vi "MC AOTF Engine.vi"(0 "Notifier Name":string, 11 "Ports (Unused)":string[](array[string])) -> ()   [LabVIEW 2016]
uses:
  AOTF Controls/AOTF Notifier Element.ctl
  AOTF Controls/AOTF Actions.ctl
  AOTF Controls/AOTF Lines Lines Control.ctl
  <vilib>/ULx/Create Channel.llb/ULx Create Channel (DO-Digital Output).vi
  <vilib>/ULx/Write.llb/ULx Write (Digital Bool 1Line 1Point).vi
  <vilib>/ULx/Create Channel.llb/ULx Create Channel (AO-Voltage-Basic).vi
  <vilib>/ULx/Write.llb/ULx Write (Analog 1D DBL 1Chan 1Samp).vi
panel:
  in  "Blank":bool
  in  "Quit":bool
  in  "500":dbl(slide) scale=0.0..100.0
  in  "642":dbl(slide) scale=0.0..100.0
  in  "560":dbl(slide) scale=0.0..100.0
  in  "488":dbl(slide) scale=0.0..100.0
  in  "405":dbl(slide) scale=0.0..100.0
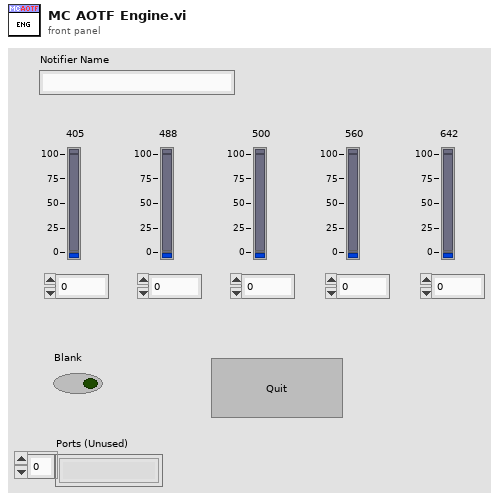
[diagram p1: front panel]
types:
  T1 = typedef "AOTF Lines Lines Control.ctl" = cluster{"Wavelength":u16[], "AO Line":string[]}
  T2 = typedef "AOTF Notifier Element.ctl" = cluster{"AOTF Action":T3, "Laser Line":string, "Power (%)":dbl, "Beam Blank On/Off":bool, "Line On/Off":bool, "Error":errorcluster, "Wavelengths (nm)":string[]}
  T3 = typedef "AOTF Actions.ctl" = enum16{"Error Check", "Blank", "Line On/Off", "Set Power", "Status", "Quit"}
  T4 = enum32{"Invalid", "Standard", "Closed", "Hidden", "Minimized", "Maximized"}
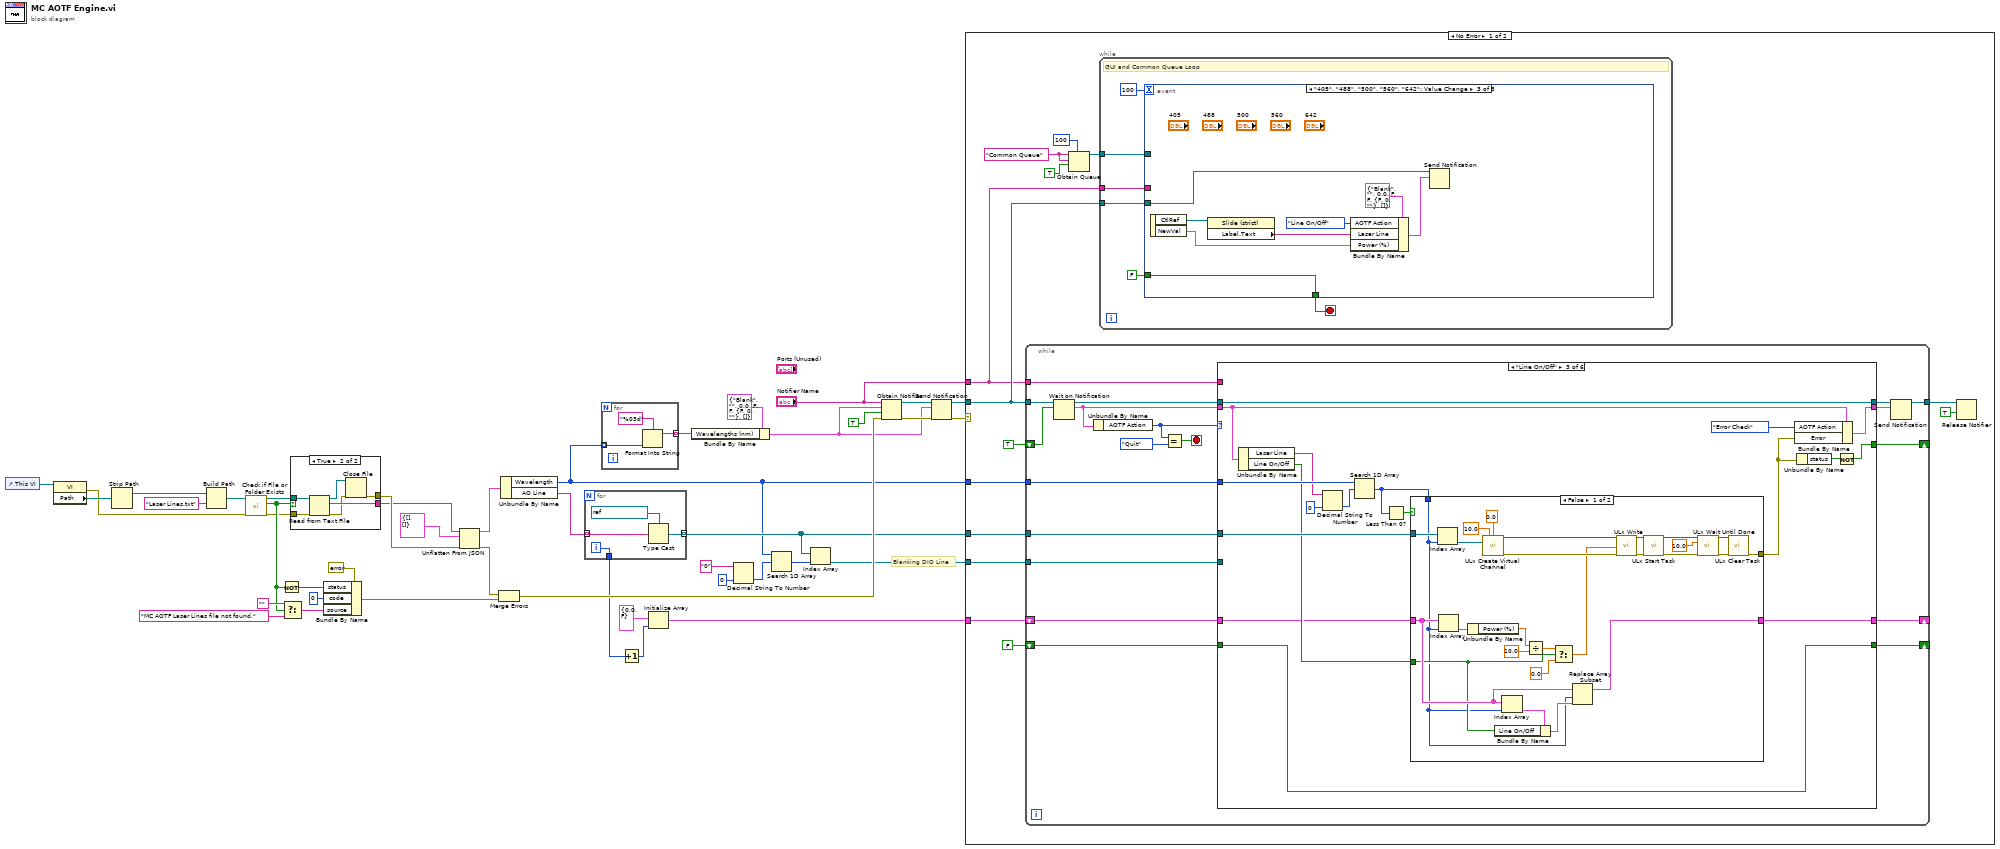
[diagram p0: block diagram]
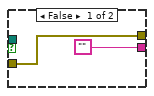
[diagram p2: hidden frame]
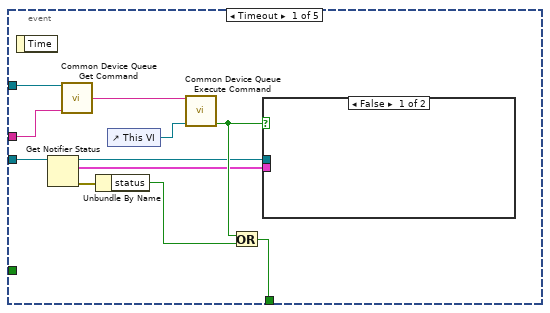
[diagram p3: hidden frame]
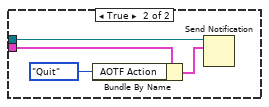
[diagram p4: hidden frame]
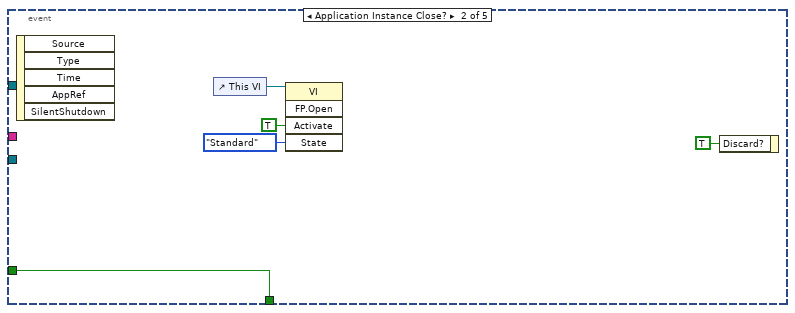
[diagram p5: hidden frame]
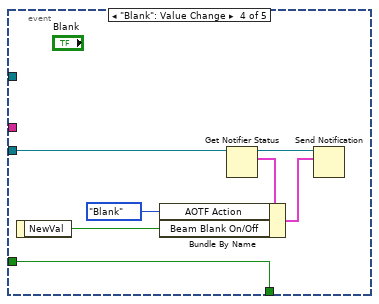
[diagram p6: hidden frame]
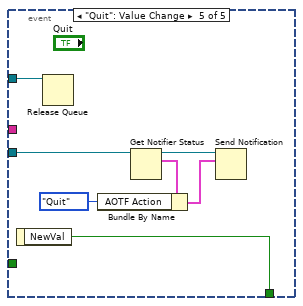
[diagram p7: hidden frame]
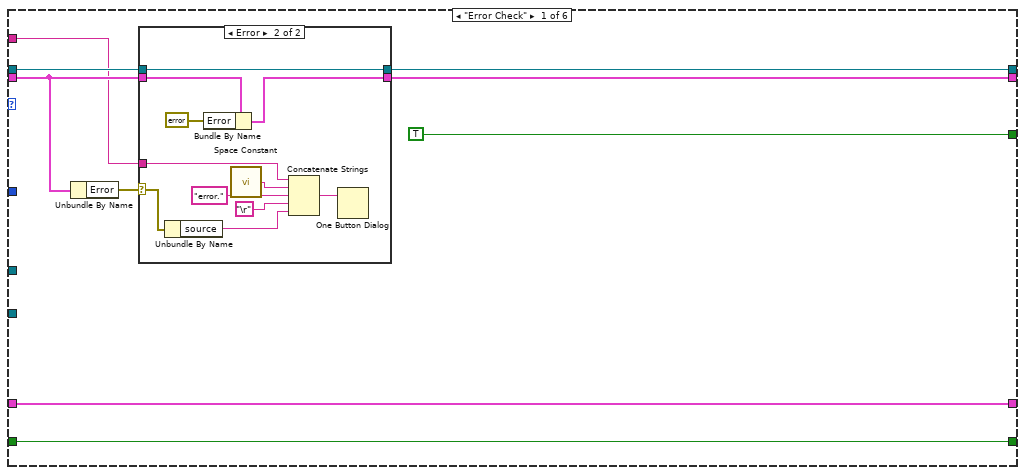
[diagram p8: hidden frame]
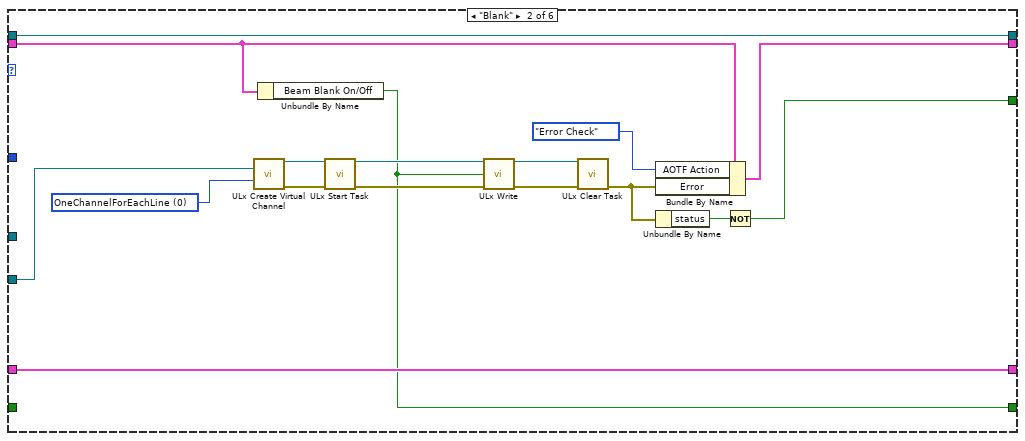
[diagram p10: hidden frame]
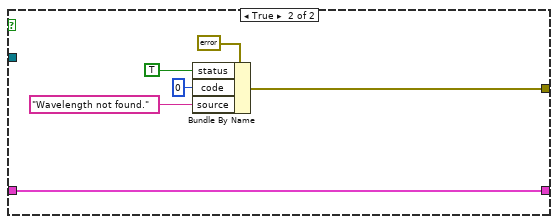
[diagram p11: hidden frame]
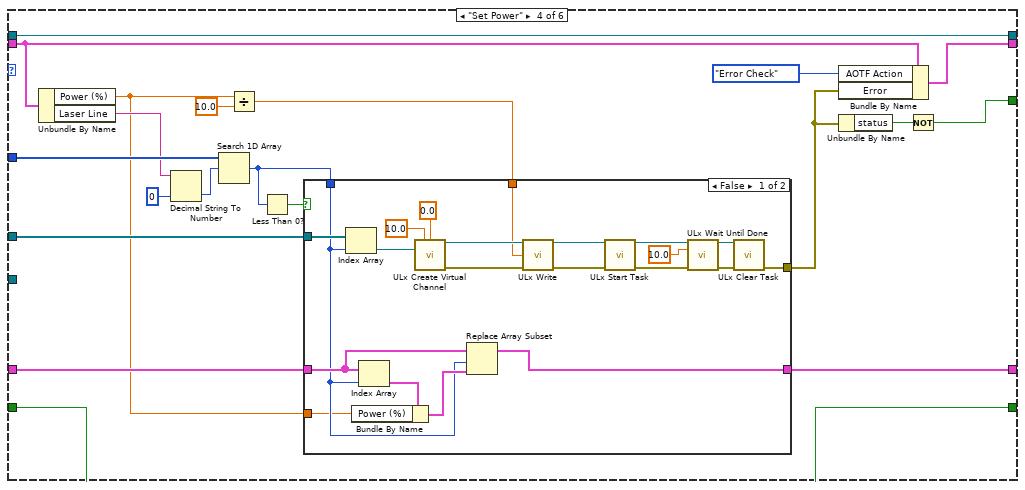
[diagram p12: hidden frame]
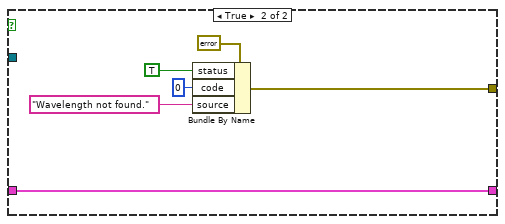
[diagram p13: hidden frame]
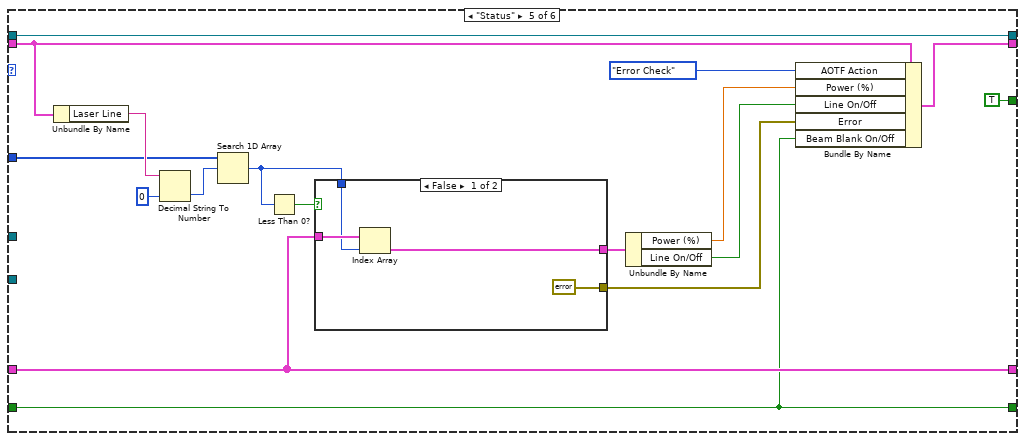
[diagram p14: hidden frame]
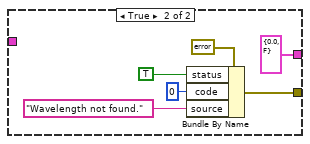
[diagram p15: hidden frame]
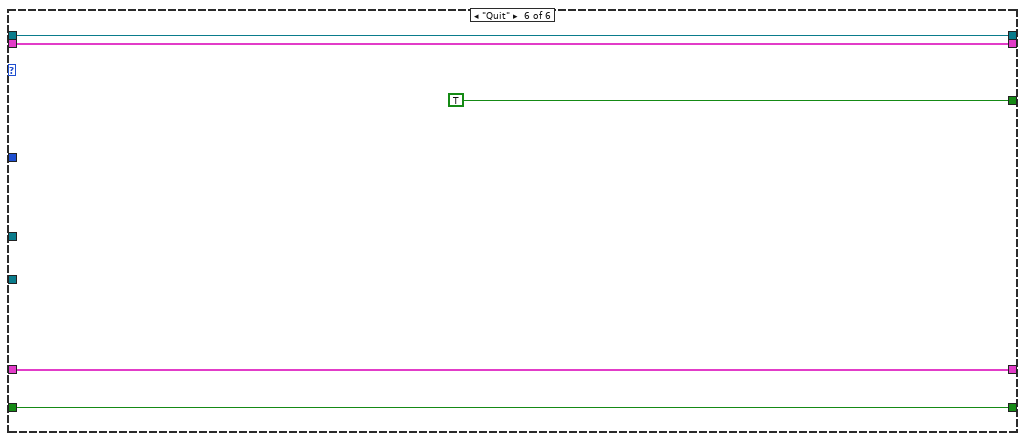
[diagram p16: hidden frame]
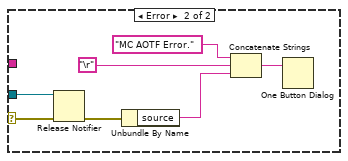
[diagram p17: hidden frame]
diagram:
  # "Blanking DIO Line"
  n1 = control-ref of="This VI"() -> (w42:refnum<vi>)
  n2 = property class="VI"(reference=w42) -> (error out=w28:errorcluster, "Path"=w41:path)  [unwired: 1 in, 1 out]
  n3 = Strip Path(path=w41) -> (stripped path=w40:path)  [unwired: 1 out]
  n4 = Build Path(base path=w40, name or relative path="Laser Lines.txt") -> (appended path=w38:path)
  n5 = call <vilib>:"Check if File or Folder Exists.vi"("error in (no error)"=w28, "path"=w38) -> ("error out"=w27:errorcluster, "file or folder exists?"=w30:bool, "dup path"=w29:path)  [unwired: 7 in]
  n6 = Not(x=w30) -> (.not. x?=w35:bool)
  n7 = Select(t="", s=w30, f="MC AOTF Laser Lines file not found." ("source")) -> (s? t:f=w31:string)
  n8 = case shown="True" w30 {
    tunnel: w29 -> [_ w51]
    tunnel: ["" w50] -> w22
    tunnel: w27 -> [w44 w48]
    tunnel: [w44 w46] -> w26
    frame False {
    }
    frame True {
      n9 = Read from Text File(file (use dialog)=w51, error in=w48) -> (refnum out=w49:refnum<file>, text=w50:string, error out=w47:errorcluster)  [unwired: 2 in, 1 out]
      n10 = Close File(refnum=w49, error in=w47) -> (error out=w46:errorcluster)  [unwired: 1 out]
    }
  }
  n11 = Bundle By Name(cluster=errorcluster {"status"=FALSE, "code"=0, "source"=""} ("Error"), "status"=w35, "code"=0, "source"=w31) -> (w24:errorcluster)
  n12 = Unflatten From JSON(JSON string=w22, type and defaults=T1 {"Wavelength"=[], "AO Line"=[]} ("Laser Lines"), error in (no error)=w26) -> (value=w20:T1, error out=w25:errorcluster)  [unwired: 4 in]
  n13 = Merge Errors(w25, w24) -> (w23:errorcluster)
  n14 = Unbundle By Name(w20) -> ("Wavelength"=w4:u16[], "AO Line"=w19:string[])
  n15 = for {
    tunnel: w19 -> [w54] mode=indexing
    tunnel: [w53] -> w15 mode=indexing
    tunnel: [w52] -> w10
    i -> [w52]
    n16 = Type Cast(type=refnum<k21> "Dev0/Ao12" ("Type Thingy"), x=w54) -> (*(type *) &x=w53:refnum<k21>)
  }
  n17 = for {
    tunnel: w4 -> [w58] mode=indexing
    tunnel: [w57] -> w2 mode=indexing
    n18 = Format Into String(format string="%03d", w58) -> (resulting string=w57:string)  [unwired: 2 in, 1 out]
  }
  n19 = Increment(x=w10) -> (x+1=w11:i32)
  n20 = Initialize Array(cluster{"Power (%)":dbl, "Line On/Off":bool} {"Power (%)"=0.0, "Line On/Off"=FALSE} ("Line Staus Cluster"), w11) -> (w9:cluster{"Power (%)":dbl, "Line On/Off":bool}[])
  n21 = Bundle By Name(cluster=T2 {"AOTF Action"=enum."Blank", "Laser Line"="", "Power (%)"=0.0, "Beam Blank On/Off"=FALSE, "Line On/Off"=FALSE, "Error"={"status"=FALSE, "code"=0, "source"=""}, "Wavelengths (nm)"=[]} ("AOTFQueueCtrl"), "Wavelengths (nm)"=w2) -> (w1:T2)
  n22 = Decimal String To Number(string="0", default (0L)=u16 0 ("default (0 I32)")) -> (number=w16:u16)  [unwired: 1 in, 1 out]
  n23 = Search 1D Array(1D array=w4, element=w16) -> (index of element=w14:i32)  [unwired: 1 in]
  n24 = Index Array(array=w15, index=w14) -> (element=w13:refnum<k21>)
  n25 = Obtain Notifier(name (unnamed)="Notifier Name", notification data type=w1, create if not found? (T)=TRUE, error in (no error)=w23) -> (notifier out=w8:refnum<notifier>, error out=w6:errorcluster)  [unwired: 1 out]
  n26 = Send Notification(notification=w1, notifier=w8, error in (no error)=w6) -> (notifier out=w7:refnum<notifier>, error out=w5:errorcluster)
  n27 = case shown="No Error" w5 {
    selector: w5 -> [_ w313]
    tunnel: w7 -> [w68 w314]
    tunnel: "Notifier Name" -> [w64 _]
    tunnel: w4 -> [w63 _]
    tunnel: w15 -> [w62 _]
    tunnel: w13 -> [w61 _]
    tunnel: w9 -> [w59 _]
    frame No Error {
      w72 = "Common Queue" ("Unique Notifier Name")
      n28 = while {
        tunnel: w68 -> [w139]
        shift-right: [w130] -> _
        shift-left: TRUE ("ignore previous (F)") -> [w138]
        tunnel: [w129] -> w66
        tunnel: w64 -> [w128]
        tunnel: w63 -> [w127]
        tunnel: w62 -> [w126]
        tunnel: w61 -> [w125]
        shift-right: [w121] -> _
        shift-left: FALSE -> [w122]
        shift-right: [w123] -> _
        shift-left: w59 -> [w124]
        stop <- w133 stop-if-true
        n29 = Wait on Notification(notifier=w139, ignore previous (F)=w138) -> (notifier out=w137:refnum<notifier>, notification=w136:T2)  [unwired: 2 in, 2 out]
        n30 = Unbundle By Name(w136) -> ("AOTF Action"=w135:T3)
        n31 = Equal?(x=w135, y=AOTF_Actions."Quit") -> (x = y?=w133:bool)
        n32 = case shown="\"Line On/Off\"" w135 {
          tunnel: w137 -> [w148 w171 w194 w246 w292 w307]
          tunnel: w136 -> [w146 w170 w187 w237 w278 w306]
          tunnel: [w144 w171 w194 w246 w292 w307] -> w132
          tunnel: [w143 w169 w186 w236 w280 w306] -> w131
          tunnel: [TRUE w165 w185 w235 TRUE TRUE] -> w130
          tunnel: w128 -> [w145 _ _ _ _ _]
          tunnel: w127 -> [_ _ w196 w248 w281 _]
          tunnel: w126 -> [_ _ w195 w247 _ _]
          tunnel: w125 -> [_ w164 _ _ _ _]
          tunnel: w124 -> [w141 w163 w180 w232 w277 w304]
          tunnel: [w141 w163 w179 w231 w277 w304] -> w123
          tunnel: w122 -> [w140 _ w181 w230 w276 w303]
          tunnel: [w140 w162 w181 w230 w276 w303] -> w121
          frame "Error Check" {
            n33 = Unbundle By Name(w146) -> ("Error"=w147:errorcluster)
            n34 = case shown="Error" w147 {
              selector: w147 -> [_ w154]
              tunnel: w146 -> [w149 w158]
              tunnel: [w150 w156] -> w144
              tunnel: w148 -> [w150 w156]
              tunnel: w145 -> [_ w153]
              tunnel: [w149 w155] -> w143
              frame No Error {
              }
              frame Error {
                n35 = Unbundle By Name(w154) -> ("source"=w152:string)
                n36 = Bundle By Name(cluster=w158, "Error"=errorcluster {"status"=FALSE, "code"=0, "source"=""}) -> (w155:T2)
                n37 = call <vilib>:"Space Constant.vi"() -> ("String"=w161:string)
                n38 = Concatenate Strings(w153, w161, "error." ("string"), "\r", w152) -> (w159:string)
                n39 = One Button Dialog(message=w159) -> ()  [unwired: 1 in, 1 out]
              }
            }
          }
          frame "Blank" {
            w172 = 0 items=["OneChannelForEachLine", "OneChannelForAllLines"] ("line grouping")
            n40 = call-poly <vilib>:"ULx Create Virtual Channel.vi"("lines"=w164, "line grouping"=w172) -> ("task out"=w173:refnum<k24>, "error out"=w174:errorcluster)  [unwired: 12 in]
            n41 = Unbundle By Name(w170) -> ("Beam Blank On/Off"=w162:bool)
            n42 = call <vilib>:"ULx Start Task.vi"("task in"=w173, "error in"=w174) -> ("task out"=w175:refnum<k24>, "error out"=w176:errorcluster)  [unwired: 12 in]
            n43 = call-poly <vilib>:"ULx Write.vi"("task in"=w175, "data"=w162, "error in"=w176) -> ("task out"=w177:refnum<k24>, "error out"=w178:errorcluster)  [unwired: 10 in, 1 out]
            n44 = call <vilib>:"ULx Clear Task.vi"("task in"=w177, "error in"=w178) -> ("error out"=w167:errorcluster)  [unwired: 13 in]
            n45 = Bundle By Name(cluster=w170, "AOTF Action"=AOTF_Actions."Error Check", "Error"=w167) -> (w169:T2)
            n46 = Unbundle By Name(w167) -> ("status"=w166:bool)
            n47 = Not(x=w166) -> (.not. x?=w165:bool)
          }
          frame "Line On/Off" {
            n48 = Unbundle By Name(w187) -> ("Laser Line"=w193:string, "Line On/Off"=w182:bool)
            n49 = Decimal String To Number(string=w193, default (0L)=u16 0 ("default (0 I32)")) -> (number=w191:u16)  [unwired: 1 in, 1 out]
            n50 = Search 1D Array(1D array=w196, element=w191) -> (index of element=w183:i32)  [unwired: 1 in]
            n51 = Less Than 0?(x=w183) -> (x < 0?=w184:bool)
            n52 = case shown="False" w184 {
              tunnel: w195 -> [w222 _]
              tunnel: [w210 w224] -> w188
              tunnel: w183 -> [w198 _]
              tunnel: w180 -> [w200 w223]
              tunnel: w182 -> [w199 _]
              tunnel: [w197 w223] -> w179
              frame False {
                n53 = Index Array(array=w222, index=w198) -> (element=w211:refnum<k21>)
                n54 = Index Array(array=w200, index=w198) -> (element=w208:cluster{"Power (%)":dbl, "Line On/Off":bool})
                n55 = Unbundle By Name(w208) -> ("Power (%)"=w205:dbl)
                n56 = call-poly <vilib>:"ULx Create Virtual Channel.vi"("maximum value"=10.0, "minimum value"=0.0, "physical channels"=w211) -> ("task out"=w221:refnum<k24>, "error out"=w214:errorcluster)  [unwired: 11 in]
                n57 = Index Array(array=w200, index=w198) -> (element=w202:cluster{"Power (%)":dbl, "Line On/Off":bool})
                n58 = Bundle By Name(cluster=w202, "Line On/Off"=w199) -> (w201:cluster{"Power (%)":dbl, "Line On/Off":bool})
                n59 = Divide(x=w205, y=10.0) -> (x/y=w204:dbl)
                n60 = Select(t=w204, s=w199, f=0.0 ("minimum value")) -> (s? t:f=w203:dbl)
                n61 = Replace Array Subset(array=w200, new element=w201, index=w198) -> (w197:cluster{"Power (%)":dbl, "Line On/Off":bool}[])
                n62 = call-poly <vilib>:"ULx Write.vi"("task in"=w221, "data"=w203, "error in"=w214) -> ("task out"=w209:refnum<k24>, "error out"=w215:errorcluster)  [unwired: 10 in, 1 out]
                n63 = call <vilib>:"ULx Start Task.vi"("task in"=w209, "error in"=w215) -> ("task out"=w220:refnum<k24>, "error out"=w217:errorcluster)  [unwired: 12 in]
                n64 = call <vilib>:"ULx Wait Until Done.vi"("task in"=w220, "timeout"=10.0, "error in"=w217) -> ("task out"=w219:refnum<k24>, "error out"=w216:errorcluster)  [unwired: 11 in]
                n65 = call <vilib>:"ULx Clear Task.vi"("task in"=w219, "error in"=w216) -> ("error out"=w210:errorcluster)  [unwired: 13 in]
              }
              frame True {
                n66 = Bundle By Name(cluster=errorcluster {"status"=FALSE, "code"=0, "source"=""} ("error out"), "status"=TRUE, "code"=0, "source"="Wavelength not found.") -> (w224:errorcluster)
              }
            }
            n67 = Bundle By Name(cluster=w187, "AOTF Action"=AOTF_Actions."Error Check", "Error"=w188) -> (w186:T2)
            n68 = Unbundle By Name(w188) -> ("status"=w189:bool)
            n69 = Not(x=w189) -> (.not. x?=w185:bool)
          }
          frame "Set Power" {
            n70 = Unbundle By Name(w237) -> ("Power (%)"=w229:dbl, "Laser Line"=w245:string)
            n71 = Decimal String To Number(string=w245, default (0L)=u16 0 ("default (0 I32)")) -> (number=w243:u16)  [unwired: 1 in, 1 out]
            n72 = Search 1D Array(1D array=w248, element=w243) -> (index of element=w233:i32)  [unwired: 1 in]
            n73 = Divide(x=w229, y=10.0) -> (x/y=w241:dbl)
            n74 = Less Than 0?(x=w233) -> (x < 0?=w234:bool)
            n75 = case shown="False" w234 {
              tunnel: w247 -> [w269 _]
              tunnel: w241 -> [w257 _]
              tunnel: [w256 w271] -> w238
              tunnel: w233 -> [w251 _]
              tunnel: w232 -> [w252 w270]
              tunnel: [w250 w270] -> w231
              tunnel: w229 -> [w249 _]
              frame False {
                n76 = Index Array(array=w269, index=w251) -> (element=w258:refnum<k21>)
                n77 = Index Array(array=w252, index=w251) -> (element=w254:cluster{"Power (%)":dbl, "Line On/Off":bool})
                n78 = Bundle By Name(cluster=w254, "Power (%)"=w249) -> (w253:cluster{"Power (%)":dbl, "Line On/Off":bool})
                n79 = call-poly <vilib>:"ULx Create Virtual Channel.vi"("maximum value"=10.0, "minimum value"=0.0, "physical channels"=w258) -> ("task out"=w268:refnum<k24>, "error out"=w261:errorcluster)  [unwired: 11 in]
                n80 = Replace Array Subset(array=w252, new element=w253, index=w251) -> (w250:cluster{"Power (%)":dbl, "Line On/Off":bool}[])
                n81 = call-poly <vilib>:"ULx Write.vi"("task in"=w268, "data"=w257, "error in"=w261) -> ("task out"=w255:refnum<k24>, "error out"=w262:errorcluster)  [unwired: 10 in, 1 out]
                n82 = call <vilib>:"ULx Start Task.vi"("task in"=w255, "error in"=w262) -> ("task out"=w267:refnum<k24>, "error out"=w264:errorcluster)  [unwired: 12 in]
                n83 = call <vilib>:"ULx Wait Until Done.vi"("task in"=w267, "timeout"=10.0, "error in"=w264) -> ("task out"=w266:refnum<k24>, "error out"=w263:errorcluster)  [unwired: 11 in]
                n84 = call <vilib>:"ULx Clear Task.vi"("task in"=w266, "error in"=w263) -> ("error out"=w256:errorcluster)  [unwired: 13 in]
              }
              frame True {
                n85 = Bundle By Name(cluster=errorcluster {"status"=FALSE, "code"=0, "source"=""} ("error out"), "status"=TRUE, "code"=0, "source"="Wavelength not found.") -> (w271:errorcluster)
              }
            }
            n86 = Bundle By Name(cluster=w237, "AOTF Action"=AOTF_Actions."Error Check", "Error"=w238) -> (w236:T2)
            n87 = Unbundle By Name(w238) -> ("status"=w239:bool)
            n88 = Not(x=w239) -> (.not. x?=w235:bool)
          }
          frame "Status" {
            n89 = Unbundle By Name(w278) -> ("Laser Line"=w284:string)
            n90 = Decimal String To Number(string=w284, default (0L)=u16 0 ("default (0 I32)")) -> (number=w283:u16)  [unwired: 1 in, 1 out]
            n91 = Search 1D Array(1D array=w281, element=w283) -> (index of element=w286:i32)  [unwired: 1 in]
            n92 = Less Than 0?(x=w286) -> (x < 0?=w285:bool)
            n93 = case shown="False" w285 {
              tunnel: w277 -> [w296 _]
              tunnel: [errorcluster {"status"=FALSE, "code"=0, "source"=""} ("error out") w298] -> w288
              tunnel: w286 -> [w295 _]
              tunnel: [w294 cluster{"Power (%)":dbl, "Line On/Off":bool} {"Power (%)"=0.0, "Line On/Off"=FALSE} ("Line Staus Cluster")] -> w289
              frame False {
                n94 = Index Array(array=w296, index=w295) -> (element=w294:cluster{"Power (%)":dbl, "Line On/Off":bool})
              }
              frame True {
                n95 = Bundle By Name(cluster=errorcluster {"status"=FALSE, "code"=0, "source"=""} ("error out"), "status"=TRUE, "code"=0, "source"="Wavelength not found.") -> (w298:errorcluster)
              }
            }
            n96 = Unbundle By Name(w289) -> ("Power (%)"=w290:dbl, "Line On/Off"=w291:bool)
            n97 = Bundle By Name(cluster=w278, "AOTF Action"=AOTF_Actions."Error Check", "Power (%)"=w290, "Line On/Off"=w291, "Error"=w288, "Beam Blank On/Off"=w276) -> (w280:T2)
          }
          frame "Quit" {
          }
        }
        n98 = Send Notification(notification=w131, notifier=w132) -> (notifier out=w129:refnum<notifier>)  [unwired: 1 in, 1 out]
      }
      n99 = Obtain Queue(max queue size (-1, unlimited)=100, name (unnamed)=w72, element data type=w72, create if not found? (T)=TRUE) -> (queue out=w69:refnum<queue>)  [unwired: 1 in, 2 out]
      n100 = while {
        tunnel: w69 -> [w77]
        tunnel: w64 -> [w75]
        tunnel: w68 -> [w76]
        stop <- w74 stop-if-true
        # "GUI and Common Queue Loop"
        n101 = event shown="[2] \"405\", \"488\", \"500\", \"560\", \"642\": Value Change" {
          selector: _ -> [_ _ _ _ _]
          dyn-events: _ -> [_ _ _ _ _]
          timeout: 100 -> [_ _ _ _ _]
          tunnel: w77 -> [w84 _ _ _ w120]
          tunnel: w76 -> [w80 _ w105 w112 w119]
          tunnel: w75 -> [w83 _ _ _ _]
          tunnel: [w82 w98 w106 w113 w117] -> w74
          tunnel: FALSE -> [_ w98 w106 w113 _]
          event Timeout {
            n102 = event-data() -> ()  [unwired: 1 in, 1 out]
            n103 = Get Notifier Status(notifier=w80) -> (notifier out=w79:refnum<notifier>, current notification=w81:T2, error out=w89:errorcluster)  [unwired: 1 in, 2 out]
            n104 = call "Common Device Queue Get Command.vi"("Common Queue"=w84, "Notifier Name"=w83) -> ("Command"=w88:string)  [unwired: 12 in, 1 out]
            n105 = Unbundle By Name(w89) -> ("status"=w86:bool)
            n106 = control-ref of="This VI"() -> (w87:refnum<vi>)
            n107 = call "Common Device Queue Execute Command.vi"("Common Command"=w88, "VI Refnum"=w87) -> ("Quit?"=w85:bool)  [unwired: 12 in, 1 out]
            n108 = Or(x=w85, y=w86) -> (x .or. y?=w82:bool)
            n109 = case shown="False" w85 {
              tunnel: w79 -> [_ w93]
              tunnel: w81 -> [_ w92]
              frame False {
              }
              frame True {
                n110 = Bundle By Name(cluster=w92, "AOTF Action"=AOTF_Actions."Quit") -> (w91:T2)
                n111 = Send Notification(notification=w91, notifier=w93) -> ()  [unwired: 1 in, 2 out]
              }
            }
          }
          event Application Instance Close? {
            n112 = event-data() -> ()  [unwired: 1 in, 5 out]
            n113 = control-ref of="This VI"() -> (w95:refnum<vi>)
            n114 = invoke class="VI" method="FP.Open"(reference=w95, "Activate"=TRUE ("Activate?"), "State"=T4."Standard") -> ()  [unwired: 2 in, 5 out]
            n115 = event-data("Discard?"=TRUE) -> ()  [unwired: 1 in, 1 out]
          }
          event "405", "488", "500", "560", "642": Value Change {
            n116 = event-data() -> ("CtlRef"=w104:refnum<vi>, "NewVal"=w100:dbl)  [unwired: 1 in]
            n117 = property class="Slide (strict)"(reference=w104) -> ("Label.Text"=w101:string)  [unwired: 1 in, 2 out]
            n118 = Bundle By Name(cluster=T2 {"AOTF Action"=enum."Blank", "Laser Line"="", "Power (%)"=0.0, "Beam Blank On/Off"=FALSE, "Line On/Off"=FALSE, "Error"={"status"=FALSE, "code"=0, "source"=""}, "Wavelengths (nm)"=[]} ("AOTFQueueCtrl"), "AOTF Action"=AOTF_Actions."Line On/Off", "Laser Line"=w101, "Power (%)"=w100) -> (w99:T2)
            n119 = Send Notification(notification=w99, notifier=w105) -> ()  [unwired: 1 in, 2 out]
          }
          event "Blank": Value Change {
            n120 = event-data() -> ("NewVal"=w108:bool)  [unwired: 1 in]
            n121 = Get Notifier Status(notifier=w112) -> (notifier out=w111:refnum<notifier>, current notification=w110:T2)  [unwired: 1 in, 3 out]
            n122 = Bundle By Name(cluster=w110, "AOTF Action"=AOTF_Actions."Blank", "Beam Blank On/Off"=w108) -> (w107:T2)
            n123 = Send Notification(notification=w107, notifier=w111) -> ()  [unwired: 1 in, 2 out]
          }
          event "Quit": Value Change {
            n124 = event-data() -> ("NewVal"=w117:bool)  [unwired: 1 in]
            n125 = Release Queue(queue=w120) -> ()  [unwired: 2 in, 3 out]
            n126 = Get Notifier Status(notifier=w119) -> (notifier out=w118:refnum<notifier>, current notification=w116:T2)  [unwired: 1 in, 3 out]
            n127 = Bundle By Name(cluster=w116, "AOTF Action"=AOTF_Actions."Quit") -> (w114:T2)
            n128 = Send Notification(notification=w114, notifier=w118) -> ()  [unwired: 1 in, 2 out]
          }
        }
      }
      n129 = Release Notifier(notifier=w66, force destroy? (F)=TRUE) -> ()  [unwired: 1 in, 3 out]
    }
    frame Error {
      n130 = Release Notifier(notifier=w314, error in (no error)=w313) -> (error out=w310:errorcluster)  [unwired: 1 in, 2 out]
      n131 = Unbundle By Name(w310) -> ("source"=w309:string)
      n132 = Concatenate Strings("MC AOTF Error.", "\r", w309) -> (w308:string)
      n133 = One Button Dialog(message=w308) -> ()  [unwired: 1 in, 1 out]
    }
  }
